vi "Cmd HO (TT).vi"(8 "error in (no error)":errorcluster caption="에러 입력(에러 없음)", 11 "ETS_EM2090 입력":refnum<class "ETS_EM2090.lvclass">) -> (0 "error out":errorcluster caption="에러 출력", 3 "ETS_EM2090 출력":refnum<class "ETS_EM2090.lvclass">)   [LabVIEW 2023, in "Turn Table and Mast.lvlib" / "ETS_EM2090.lvclass"]
uses:
  ETS_EM2090.lvclass
  ETS_EM2090.lvclass/ETS_EM2090.ctl
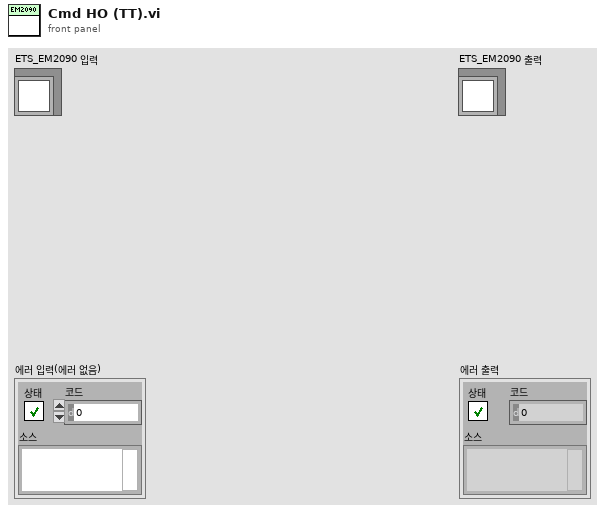
[diagram p1: front panel]
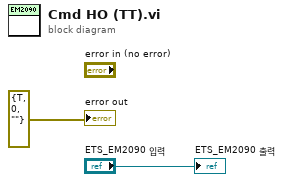
[diagram p0: block diagram]
diagram:
  "error out" <- errorcluster {"status"=TRUE, "code"=0, "source"=""} ("error out")
  "ETS_EM2090 출력" <- "ETS_EM2090 입력"
